vi "AutoDataToString.vi"(10 "File Path Name":string[](array[string]), 11 "Auto":T1) -> (3 "String":string)   [LabVIEW 2017]
uses:
  AutoFileDataType.ctl
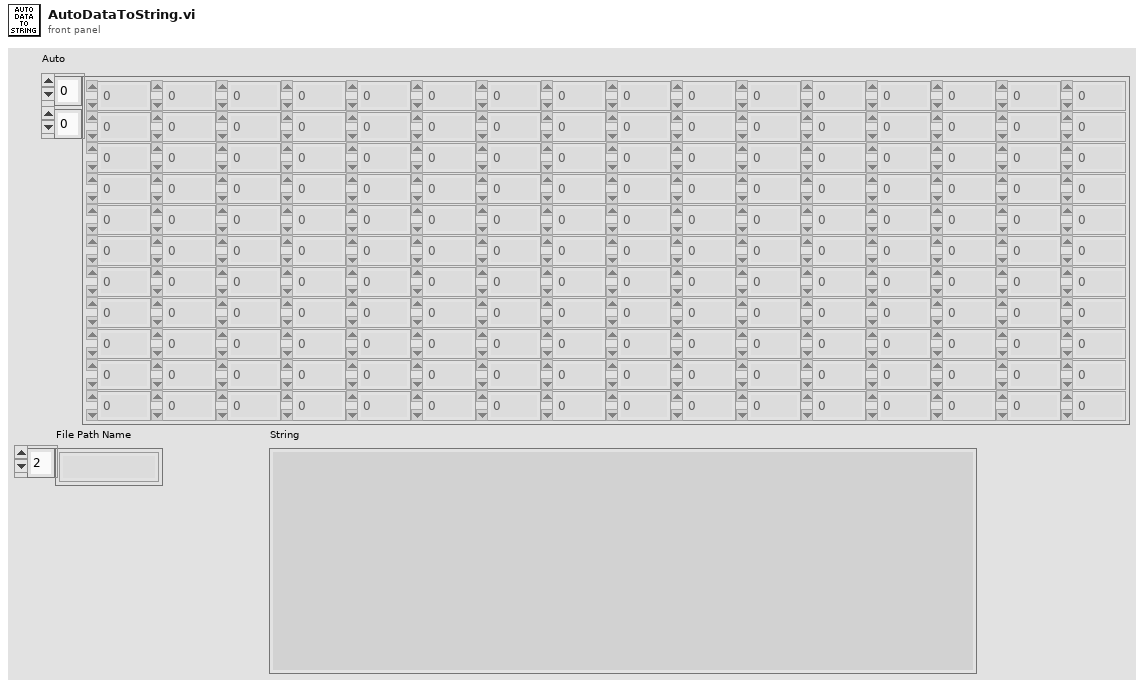
[diagram p1: front panel]
types:
  T1 = typedef "AutoFileDataType.ctl" = dbl[][]
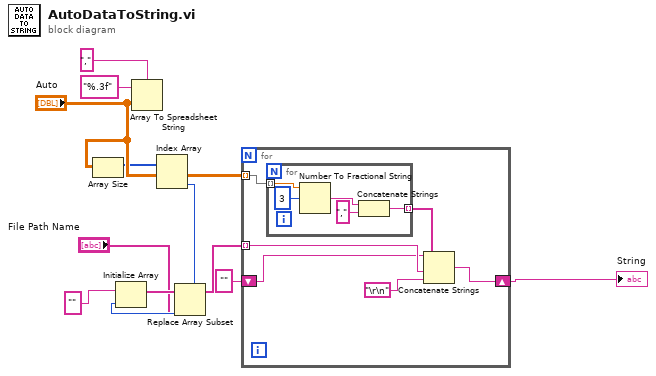
[diagram p0: block diagram]
diagram:
  n1 = Array Size(array="Auto") -> (size(s)=w5:i32[])
  n2 = Array To Spreadsheet String(delimiter (Tab)=",", array="Auto", 3:"%.3f" ("format string")) -> ()  [unwired: 1 out]
  n3 = Index Array(array=w5) -> (element #2=w4:i32)  [unwired: 2 in, 1 out]
  n4 = Initialize Array("", w4) -> (w3:string[])
  n5 = Replace Array Subset(array=w3, new element="File Path Name") -> (w1:string[])  [unwired: 1 in]
  n6 = for {
    tunnel: "Auto" -> [w17] mode=indexing
    tunnel: w1 -> [w15] mode=indexing
    shift-right: [w13] -> w8
    shift-left: "" -> [w12]
    n7 = for {
      tunnel: w17 -> [w22] mode=indexing
      tunnel: [w19] -> w16 mode=indexing
      n8 = Number To Fractional String(number=w22, precision (6)=i16 3) -> (F-format string=w21:string)  [unwired: 2 in]
      n9 = Concatenate Strings(w21, "," ("string")) -> (w19:string)
    }
    n10 = Concatenate Strings(w12, w16, w15, "\r\n") -> (w13:string)
  }
  "String" <- w8
